vi "Run Main Loop.vi"(8 "error in (no error)":errorcluster, 10 "Repeat?":bool=TRUE, 11 "DAQ Timed SPIM in":refnum<class "DAQ Timed SPIM.lvclass">) -> (0 "error out":errorcluster, 3 "DAQ Timed SPIM out":refnum<class "DAQ Timed SPIM.lvclass">)   [LabVIEW 2020, in "DAQ Timed SPIM.lvlib" / "DAQ Timed SPIM.lvclass"]
uses:
  DAQ Timed SPIM.lvclass
  C:/Program Files/National Instruments/LabVIEW 2020/vi.lib/ActorFramework/Actor/Actor.lvclass
  DAQ Timed SPIM.lvclass/DAQ Timed SPIM.ctl
  <vilib>/ActorFramework/Message Enqueuer/Message Priority.ctl
  <vilib>/ActorFramework/Actor/Actor.lvclass/Actor.ctl
  <vilib>/ActorFramework/Message Enqueuer/Message Enqueuer.lvclass/Message Enqueuer.ctl
  DAQ Timed SPIM Messages/Run Main Loop Msg/Run Main Loop Msg.lvclass/Run Main Loop Msg.ctl
  <vilib>/DAQmx/write.llb/DAQmx Write (Digital 2D U8 NChan NSamp).vi
  <vilib>/DAQmx/write.llb/DAQmx Write (Analog 2D DBL NChan NSamp).vi
  <vilib>/ActorFramework/Message Enqueuer/Init from Existing Queue.vi
  <vilib>/ActorFramework/Message Enqueuer/Enqueue.vi
  DAQ Timed SPIM Messages/Stop Triggered Acq Msg/Stop Triggered Acq Msg.lvclass
  C:/Program Files/National Instruments/LabVIEW 2020/vi.lib/ActorFramework/Message/Message.lvclass
  DAQ Timed SPIM Messages/Run Main Loop Msg/Run Main Loop Msg.lvclass
  <vilib>/DAQmx/miscellaneous.llb/DAQmx Fill In Error Info.vi
  <vilib>/ActorFramework/Message Priority Queue/Priority Enqueue.vi
  <vilib>/ActorFramework/Message Enqueuer/Message Enqueuer.lvclass
  <vilib>/ActorFramework/Actor/Actor.lvclass
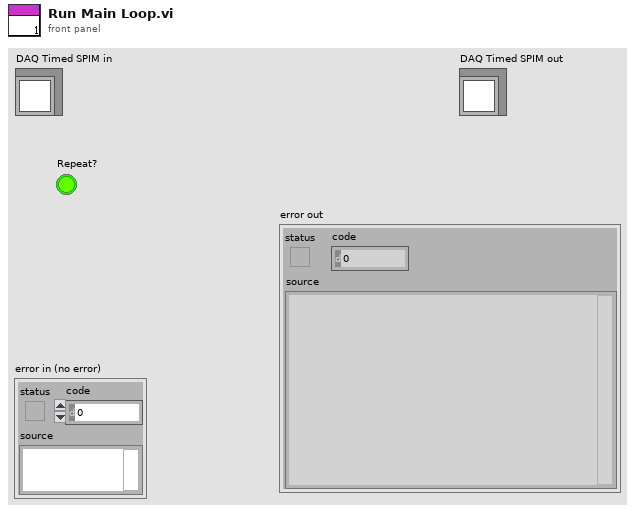
[diagram p1: front panel]
types:
  T1 = typedef "Actor Framework.lvlib/Message Enqueuer.lvclass/Message Priority.ctl" = enum16{"Low", "Normal", "High"}
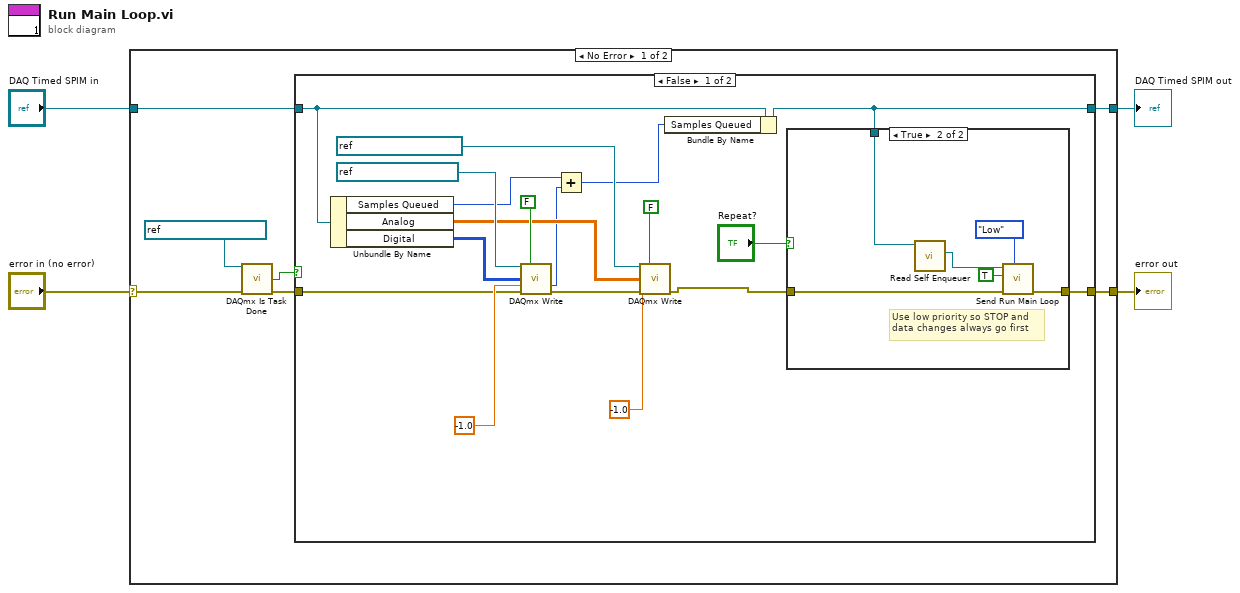
[diagram p0: block diagram]
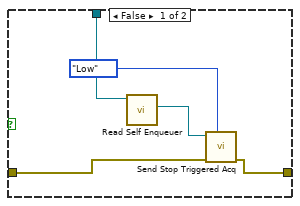
[diagram p2: hidden frame]
diagram:
  n1 = case shown="No Error" "error in (no error)" {
    selector: "error in (no error)" -> [w9 w44]
    tunnel: [w10 w44] -> w3
    tunnel: [w5 w43] -> w1
    tunnel: "DAQ Timed SPIM in" -> [w6 w43]
    frame No Error {
      n2 = call <vilib>:"DAQmx Is Task Done.vi"("task/channels in"=refnum<k21> "SPIM_Digital_Task", "error in"=w9) -> ("task done?"=w7:bool, "error out"=w8:errorcluster)  [unwired: 11 in, 1 out]
      n3 = case shown="False" w7 {
        tunnel: w8 -> [w19 w42]
        tunnel: [w23 w42] -> w10
        tunnel: w6 -> [w22 w41]
        tunnel: [w16 w41] -> w5
        frame False {
          n4 = Unbundle By Name(w22) -> ("Samples Queued"=w14:u32, "Analog"=w15:dbl[][], "Digital"=w29:u8[][])
          n5 = call-poly <vilib>:"DAQmx Write.vi"("task/channels in"=refnum<k21> "SPIM_Digital_Task", "auto start"=FALSE, "data"=w29, "timeout"=-1.0, "error in"=w19) -> ("number of samples written per channel"=w13:u32, "error out"=w18:errorcluster)  [unwired: 8 in, 1 out]
          n6 = Add(x=w14, y=w13) -> (x+y=w12:u32)
          n7 = call-poly <vilib>:"DAQmx Write.vi"("task/channels in"=refnum<k21> "SPIM_Analog_Task", "auto start"=FALSE, "data"=w15, "timeout"=-1.0, "error in"=w18) -> ("error out"=w17:errorcluster)  [unwired: 8 in, 2 out]
          n8 = Bundle By Name(cluster=w22, "Samples Queued"=w12) -> (w16:refnum<class "DAQ Timed SPIM.lvclass">)
          n9 = case shown="True" "Repeat?" {
            tunnel: w17 -> [w33 w40]
            tunnel: [w32 w39] -> w23
            tunnel: w16 -> [w34 w37]
            frame False {
              n10 = call <vilib>:"Read Self Enqueuer.vi"("Actor"=w34) -> ("Self Enqueuer"=w31:refnum<class "Message Enqueuer.lvclass">)  [unwired: 10 in]
              n11 = call "Send Stop Triggered Acq.vi"("Message Priority (Normal)"=Message_Priority."Low", "error in (no error)"=w33, "Message Enqueuer"=w31) -> ("error out"=w32:errorcluster)  [unwired: 7 in, 1 out]
            }
            frame True {
              # "Use low priority so STOP and\ndata changes always go first"
              n12 = call <vilib>:"Read Self Enqueuer.vi"("Actor"=w37) -> ("Self Enqueuer"=w36:refnum<class "Message Enqueuer.lvclass">)  [unwired: 10 in]
              n13 = call "Send Run Main Loop.vi"("Message Priority (Normal)"=Message_Priority."Low", "error in (no error)"=w40, "Repeat?"=TRUE, "Message Enqueuer"=w36) -> ("error out"=w39:errorcluster)  [unwired: 6 in, 1 out]
            }
          }
        }
        frame True {
        }
      }
    }
    frame Error {
    }
  }
  "error out" <- w3
  "DAQ Timed SPIM out" <- w1
